vi "Run.vi"(8 "error in (no error)":errorcluster, 10 "UI Refs":T1, 11 "H1FR":refnum<class "H1 Frequency Response.lvclass">) -> (0 "error out":errorcluster, 3 "H1FR out":refnum<class "H1 Frequency Response.lvclass">)   [LabVIEW 2025, in "H1 Plotter.lvlib" / "H1 Frequency Response.lvclass"]
uses:
  H1 Frequency Response.lvclass
  H1 Frequency Response.lvclass/H1 Frequency Response.ctl
  Users/Public/Documents/Sandia National Labs/TSS Plugin/Tests/XY Plotter.lvlibp/XY Plotter configuration/Read XY Plotter.vi
  Users/Public/Documents/Sandia National Labs/TSS Plugin/CEF.lvlibp/serializable configuration/CEF_serializable configuration.lvclass
  Users/Public/Documents/Sandia National Labs/TSS Plugin/Tests/XY Plotter.lvlibp/XY  Plotter/XY Plotter.lvclass
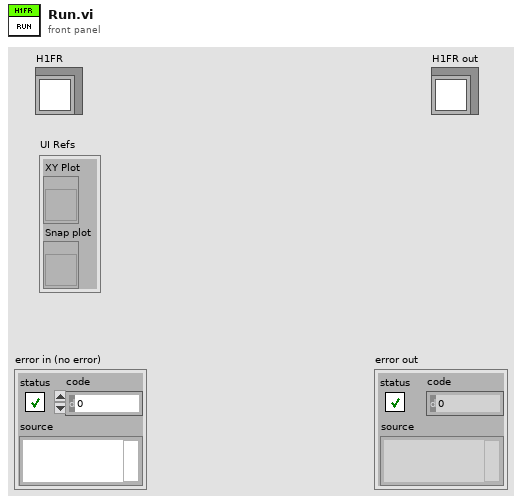
[diagram p1: front panel]
types:
  T1 = cluster{"XY Plot":refnum<vi>, "Snap plot":refnum<vi>}
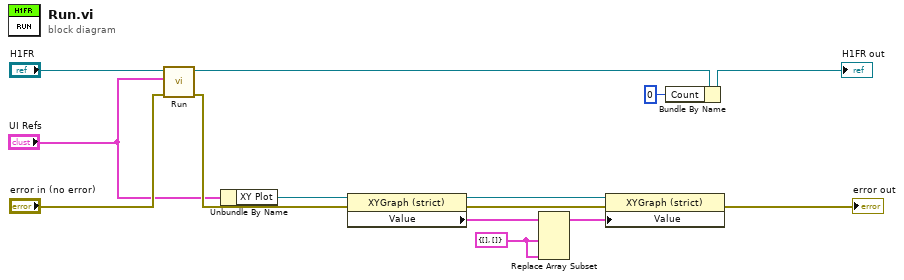
[diagram p0: block diagram]
diagram:
  w12 = cluster{"Wavenumber":dbl[], "Data":dbl[]} {"Wavenumber"=[], "Data"=[]} ("Spectrum")
  n1 = call-parent "Run.vi"("error in (no error)"="error in (no error)", "UI Refs"="UI Refs", "XY Plotter"="H1FR") -> ("error out"=w6:errorcluster, "XY Plotter out"=w14:refnum<class "H1 Frequency Response.lvclass">)  [unwired: 7 in]
  n2 = Unbundle By Name("UI Refs") -> ("XY Plot"=w1:refnum<vi>)
  n3 = property class="XYGraph (strict)"(reference=w1, error in=w6) -> (reference out=w10:refnum<vi>, error out=w5:errorcluster, "Value"=w11:cluster{"Wavenumber":dbl[], "Data":dbl[]}[])
  n4 = Replace Array Subset(array=w11, new element #1=w12, new element #2=w12) -> (w9:cluster{"Wavenumber":dbl[], "Data":dbl[]}[])  [unwired: 2 in]
  n5 = property class="XYGraph (strict)"(reference=w10, error in=w5, "Value"=w9) -> (error out=→"error out":errorcluster)  [unwired: 1 out]
  n6 = Bundle By Name(cluster=w14, "Count"=0) -> (→"H1FR out":refnum<class "H1 Frequency Response.lvclass">)
